vi "_Subsystem_Name Controller.vi"(8 "error in":errorcluster) -> ()   [LabVIEW 2023]
doc: "This VI responds to drive commands both auto and tele Opmodes.\nIt owns the drivebase motors and sensors and runs independent from opModes. Commands can run for arbitrary times, but newly posted commands will interupt as long as Check is called and used for time delays."
uses:
  Implementation/_Subsystem_Name Operations.ctl
  Implementation/_Subsystem_Name Setpoints.ctl
  <vilib>/REVLibDriver/REVLibDriver.lvlib
  <resource>/objmgr/REVSpark.rc
  <vilib>/MRC/Types/CmdCtl Completion.ctl
  <vilib>/Rock Robotics/WPI/RobotDrive/WPI_RobotDriveMecanumDrive_Cartesian.vi
  <vilib>/REV Custom Controls/REVSparkRefnum.ctl
  <vilib>/Rock Robotics/WPI/RobotDrive/WPI_RobotDriveDevRef.ctl
  <vilib>/Rock Robotics/WPI/RobotDrive/WPI_RobotDriveMecanumDrive_Polar.vi
  <vilib>/Rock Robotics/WPI/Framework/Completion Status.ctl
panel:
  out "Waveform Chart":dbl[](graph)
  in  "Abort Cmd":bool
  in  "Execute Cmd":bool
  in  "Interactive Values":T1
  out "Command Timing":cluster{"Start Time (ms)":u32, "Iterations":i32}
  out "Status":T3
  out "Current Command Data":T1
  out "Cmd Summary":string
  # "The panel for a subsystem is a great place to chart or view operational\nstate of the mechanism. You can also introduce debug-specific operations\nsuch as tuning PID or calibration."
  # "Interactive Command: You may fill in the settings for a command\nand schedule it with the Execute button. You can observe and abort\nany command while fine tuning the code for the controller."
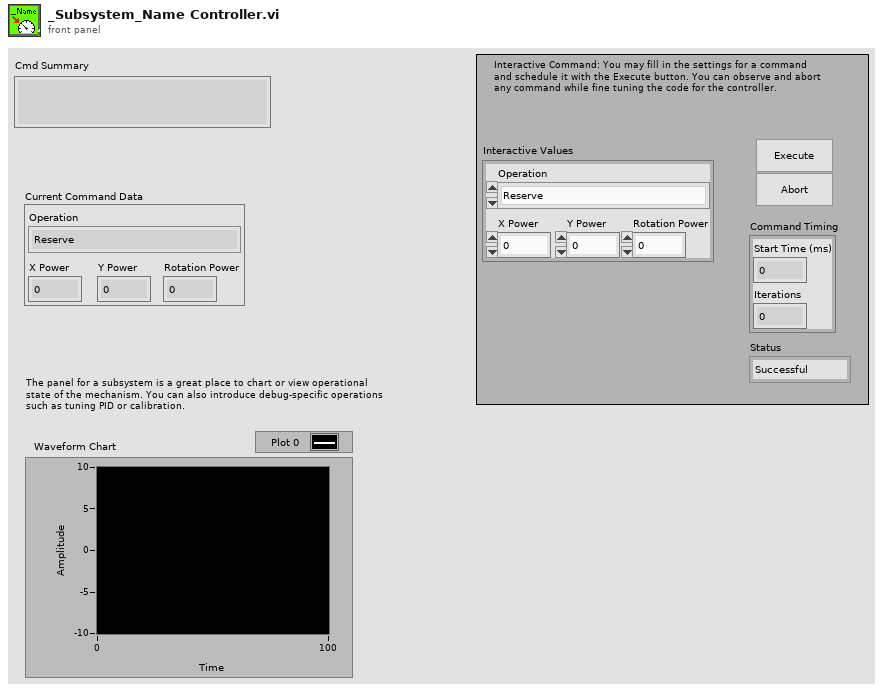
[diagram p1: front panel]
types:
  T1 = typedef "_Subsystem_Name Setpoints.ctl" = cluster{"Operation":T2, "X Power":dbl, "Y Power":dbl, "Rotation Power":dbl}
  T2 = typedef "_Subsystem_Name Operations.ctl" = enum16{"Reserve", "Read Current", "Immediate"}
  T3 = typedef "Completion Status.ctl" = enum16{"Successful", "Aborted", "Incomplete"}
  T4 = typedef "WPI_RobotDriveDevRef.ctl" = cluster{"Motors[]":T5[], "Square Inputs":bool, "Max Output":dbl}
  T5 = typedef "REVLibDriver.lvlib/REVSparkRefnum.ctl" = refnum<k20>
  T6 = cluster{"left rear":i32, "right rear":i32, "left front":i32, "right front":i32}
  T7 = typedef "Command Status Info.ctl" = cluster{"Name":string, "Status":T3, "notifier out":T8}
  T8 = typedef "Completion Notifier.ctl" = refnum<notifier>
  T9 = cluster{"Current Command":T1, "Command Timing":cluster{"Start Time (ms)":u32, "Iterations":i32}, "Command Arguments":cluster{"Command Info":T7, "Description":string, "Default Command":T1, "queue out":refnum<queue>, "Subsystem Name":string}}
  T10 = typedef "CmdCtl Completion.ctl" = enum16{"incomplete", "finished"}
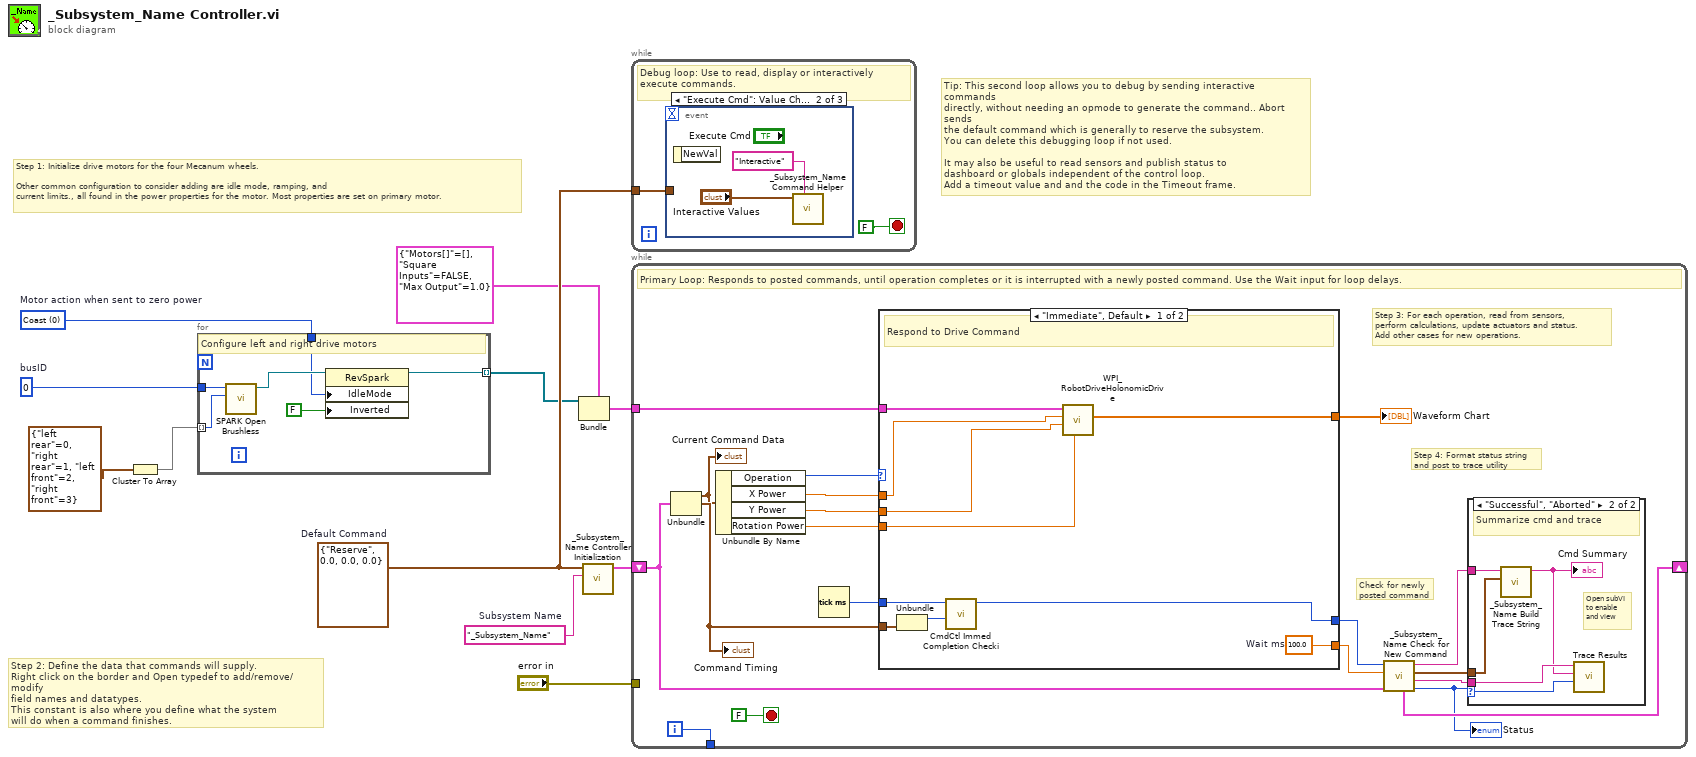
[diagram p0: block diagram]
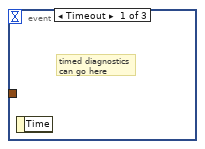
[diagram p2: hidden frame]
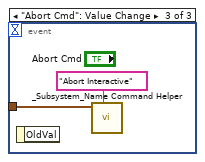
[diagram p3: hidden frame]
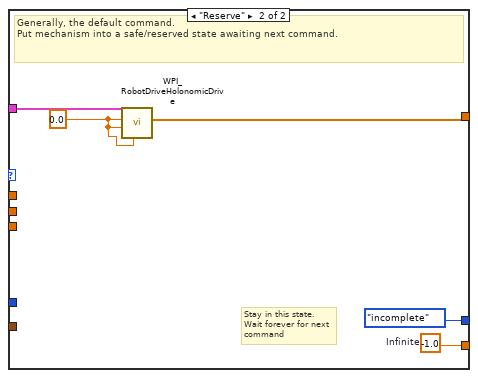
[diagram p5: hidden frame]
diagram:
  w7 = 0  # busID
  w8 = u32 0 items=["Coast", "Brake"]  # Motor action when sent to zero power
  w6 = T1 {"Operation"=enum."Reserve", "X Power"=0.0, "Y Power"=0.0, "Rotation Power"=0.0}  # Default Command
  w9 = "_Subsystem_Name"  # Subsystem Name
  # "Tip: This second loop allows you to debug by sending interactive commands\ndirectly, without needing an opmode to generate the command.. Abort sends\nthe default command which is generally to reserve the subsystem.\nYou can delete this debugging loop if not used.\n\nIt may also be useful to read sensors and publish status to\ndashboard or globals independent of the control loop.\nAdd a timeout value and and the code in the Timeout frame."
  # "Step 2: Define the data that commands will supply.\nRight click on the border and Open typedef to add/remove/modify\nfield names and datatypes.\nThis constant is also where you define what the system\nwill do when a command finishes."
  # "Step 1: Initialize drive motors for the four Mecanum wheels.\n\nOther common configuration to consider adding are idle mode, ramping, and\ncurrent limits., all found in the power properties for the motor. Most properties are set on primary motor."
  n1 = Cluster To Array(cluster=T6 {"left rear"=0, "right rear"=1, "left front"=2, "right front"=3}) -> (array=w4:i32[])
  n2 = for {
    tunnel: w8 -> [w16]
    tunnel: w7 -> [w15]
    tunnel: w4 -> [w14] mode=indexing
    tunnel: [w13] -> w3 mode=indexing
    # "Configure left and right drive motors"
    n3 = call <vilib>:"SPARK Open Brushless.vi"("deviceId"=w14, "busID"=w15) -> ("Spark refnum"=w17:T5)  [unwired: 8 in, 1 out]
    n4 = property class="RevSpark"(reference=w17, "IdleMode"=w16, "Inverted"=FALSE) -> (reference out=w13:T5)  [unwired: 1 in, 1 out]
  }
  n5 = Bundle(cluster=T4 {"Motors[]"=[], "Square Inputs"=FALSE, "Max Output"=1.0} ("RobotDriveDevRef"), "Motors[]"=w3) -> (w1:T4)  [unwired: 2 in]
  n6 = call "_Subsystem_Name Controller Initialization.vi"("Subsystem Name"=w9, "Default Command"=w6) -> ("Current Command"=w10:T9)  [unwired: 9 in]
  n7 = while {
    tunnel: w6 -> [w18]
    stop <- FALSE stop-if-true
    # "Debug loop: Use to read, display or interactively execute commands."
    n8 = event shown="[1] \"Execute Cmd\": Value Change" {
      selector: _ -> [_ _ _]
      dyn-events: _ -> [_ _ _]
      timeout: _ -> [_ _ _]
      tunnel: w18 -> [_ _ w23]
      event Timeout {
        # "timed diagnostics\ncan go here"
        # "Insert Text Here"
        n9 = event-data() -> ()  [unwired: 1 in, 1 out]
      }
      event "Execute Cmd": Value Change {
        # "Execute"
        n10 = event-data() -> ()  [unwired: 1 in, 1 out]
        n11 = call "_Subsystem_Name Command Helper.vi"("Description"="Interactive", "SubSystem Data"="Interactive Values") -> ()  [unwired: 7 in, 3 out]
      }
      event "Abort Cmd": Value Change {
        # "Insert Text Here"
        n12 = event-data() -> ()  [unwired: 1 in, 1 out]
        n13 = call "_Subsystem_Name Command Helper.vi"("Description"="Abort Interactive", "SubSystem Data"=w23) -> ()  [unwired: 7 in, 3 out]
      }
    }
  }
  n14 = while {
    shift-right: [w36] -> _
    shift-left: w10 -> [w30]
    tunnel: [w41] -> _
    tunnel: "error in" -> [_]
    tunnel: w1 -> [w25]
    i -> [w41]
    stop <- FALSE stop-if-true
    # "Step 4: Format status string\nand post to trace utility"
    # "Check for newly\nposted command"
    # "Step 3: For each operation, read from sensors,\nperform calculations, update actuators and status.\nAdd other cases for new operations."
    # "Primary Loop: Responds to posted commands, until operation completes or it is interrupted with a newly posted command. Use the Wait input for loop delays."
    n15 = Unbundle(w30) -> ("Current Command"=w28:T1, "Command Timing"=w29:cluster{"Start Time (ms)":u32, "Iterations":i32})  [unwired: 1 out]
    "Command Timing" <- w29
    "Current Command Data" <- w28
    n16 = Unbundle By Name(w28) -> ("Operation"=w40:T2, "X Power"=w39:dbl, "Y Power"=w37:dbl, "Rotation Power"=w26:dbl)
    n17 = Tick Count (ms)() -> (millisecond timer value=w38:u32)
    n18 = case shown="\"Immediate\", Default" w40 {
      tunnel: [w57 w62] -> w34
      tunnel: [w54 CmdCtl_Completion."incomplete"] -> w35
      tunnel: w29 -> [w56 _]
      tunnel: w39 -> [w51 _]
      tunnel: w38 -> [w55 _]
      tunnel: w37 -> [w50 _]
      tunnel: w26 -> [w49 _]
      tunnel: w25 -> [w52 w60]
      tunnel: [w48 w58] -> w24
      frame "Immediate", Default {
        w57 = 100.0  # Wait ms
        # "Respond to Drive Command"
        n19 = Unbundle(w56) -> ("Start Time (ms)"=w53:u32)  [unwired: 1 out]
        n20 = call <vilib>:"CmdCtl Immed Completion Checki.vi"("Start Time (ms)"=w53, "current time (ms)"=w55) -> ("Completion"=w54:T10)  [unwired: 9 in]
        n21 = call-poly <vilib>:"WPI_RobotDriveHolonomicDrive.vi"("Rotation"=w49, "Y"=w50, "X"=w51, "RobotDriveDevRef"=w52) -> ("Motor Values"=w48:dbl[])  [unwired: 5 in, 2 out]
      }
      frame "Reserve" {
        w59 = 0.0 ("X")
        w62 = -1.0  # Infinite
        # "Stay in this state.\nWait forever for next\ncommand"
        # "Generally, the default command.\nPut mechanism into a safe/reserved state awaiting next command."
        n22 = call-poly <vilib>:"WPI_RobotDriveHolonomicDrive.vi"("Rotation"=w59, "Direction"=w59, "Magnitude"=w59, "RobotDriveDevRef"=w60) -> ("Motor Values"=w58:dbl[])  [unwired: 5 in, 2 out]
      }
    }
    "Waveform Chart" <- w24
    n23 = call "_Subsystem_Name Check for New Command.vi"("Current Command"=w30, "Wait time (ms)"=w34, "Completion"=w35) -> ("Completion"=w27:T3, "Subsystem Name"=w31:string, "Current Command"=w32:T1, "Initial Trace String"=w33:string, "NextCommand"=w36:T9)  [unwired: 4 in]
    "Status" <- w27
    n24 = case shown="\"Successful\", \"Aborted\"" w27 {
      selector: w27 -> [_ w47]
      tunnel: w33 -> [_ w45]
      tunnel: w32 -> [_ w44]
      tunnel: w31 -> [_ w46]
      frame "Incomplete", Default {
        # "Continuing current command"
      }
      frame "Successful", "Aborted" {
        # "Open subVI\nto enable\nand view"
        # "Summarize cmd and trace"
        n25 = call "_Subsystem_Name Build Trace String.vi"("Current Command"=w44, "Initial Trace String"=w45) -> ("Trace String"=w43:string)  [unwired: 9 in]
        "Cmd Summary" <- w43
        n26 = call <vilib>:"Trace Results.vi"("Status of previous command"=w47, "Description"=w43, "Subsystem"=w46) -> ()  [unwired: 9 in]
      }
    }
  }
